vi "Coefficient-FGV.vi"(7 "枚举":enum16{"R", "W"}(ring), 9 "Broad":T1, 10 "机台":T2, 11 "dataIN":string[][](array[string])=[["", "5658"]]) -> (2 "Coefficient":string[](array[string]), 3 "data":string[][](array[string]))   [LabVIEW 2025, in "Coefficient.lvclass"]
uses:
  Coefficient.lvclass
  Computer.ctl
  Broad.ctl
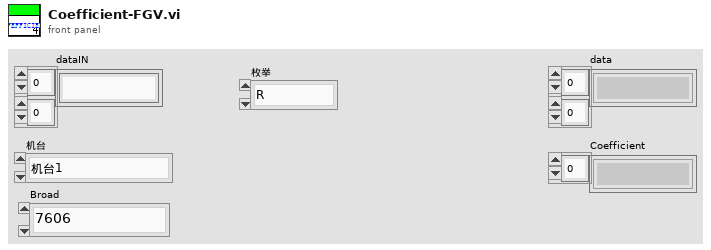
[diagram p1: front panel]
types:
  T1 = typedef "Coefficient.lvclass/Broad.ctl" = enum16{"7606", "7616"}
  T2 = typedef "Coefficient.lvclass/Computer.ctl" = enum16{"机台1", "机台2", "机台3", "备用1", "备用2", "备用3"}
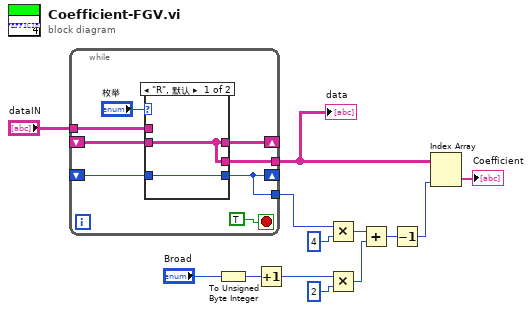
[diagram p0: block diagram]
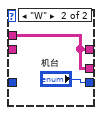
[diagram p2: hidden frame]
diagram:
  n1 = while {
    shift-right: [w18] -> _
    shift-left: _ -> [w17]
    tunnel: "dataIN" -> [w19]
    tunnel: [w16] -> w12
    shift-right: [w14] -> _
    shift-left: _ -> [w15]
    tunnel: [w14] -> w1
    stop <- TRUE stop-if-true
    n2 = case shown="\"R\", 默认" "枚举" {
      tunnel: w19 -> [_ w25]
      tunnel: [w23 w25] -> w18
      tunnel: w17 -> [w23 _]
      tunnel: [w23 w25] -> w16
      tunnel: [w22 "机台"] -> w14
      tunnel: w15 -> [w22 _]
      frame "R", Default {
      }
      frame "W" {
      }
    }
  }
  "data" <- w12
  n3 = To Unsigned Byte Integer(number="Broad") -> (unsigned 8bit integer=w3:u8)
  n4 = Increment(x=w3) -> (x+1=w7:u8)
  n5 = Multiply(x=w1, y=4) -> (x*y=w9:i32)
  n6 = Multiply(x=w7, y=2) -> (x*y=w6:i32)
  n7 = Add(x=w9, y=w6) -> (x+y=w8:i32)
  n8 = Decrement(x=w8) -> (x-1=w2:i32)
  n9 = Index Array(array=w12, index (col)=w2) -> (element=→"Coefficient":string[])  [unwired: 1 in]
